vi "AssertEqual_Tests.vi"(11 "error in":errorcluster) -> (15 "error out":errorcluster)   [LabVIEW 2016, in "DronaTest.lvlib"]
uses:
  DronaTest.lvlib
  APIs/Assert/AssertControlValue/Equal.vi
  <vilib>/addons/_JKI Toolkits/Caraya/classes/Assert/Assert Equal Value_Variant.vi
  <vilib>/addons/_JKI Toolkits/Caraya/classes/Assert/Assert Error.vi
  <vilib>/addons/_JKI Toolkits/Caraya/classes/Test/Test.lvclass
  Drona.lvlib
  <vilib>/addons/_JKI Toolkits/Caraya/classes/Assert/Assert.lvclass
  APIs/Assert/AssertControlValue/AssertControlValue.lvlib
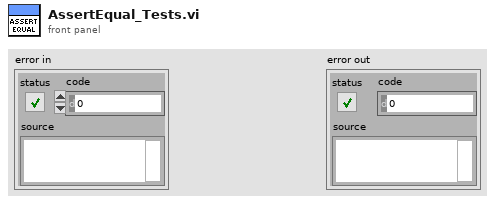
[diagram p1: front panel]
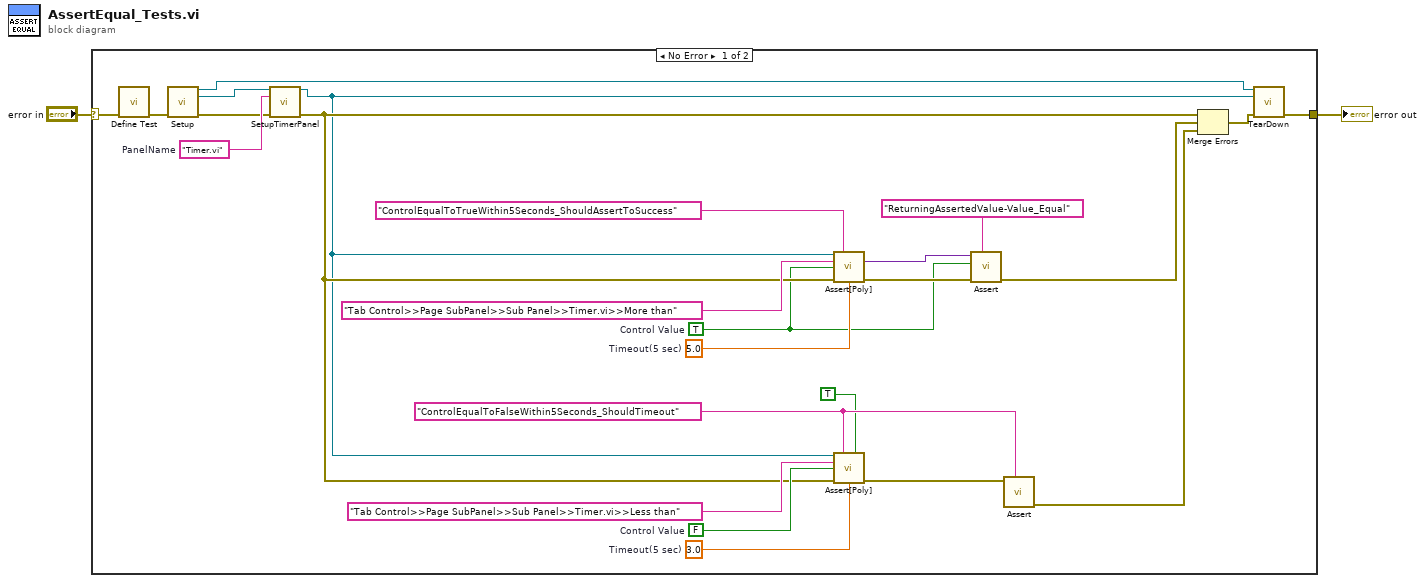
[diagram p0: block diagram]
diagram:
  n1 = case shown="No Error" "error in" {
    selector: "error in" -> [w27 w28]
    tunnel: [w12 w28] -> w1
    frame No Error {
      w17 = "Timer.vi"  # PanelName
      w26 = FALSE  # Control Value
      w23 = 3.0  # Timeout(5 sec)
      w22 = "ControlEqualToFalseWithin5Seconds_ShouldTimeout" ("string")
      w24 = 5.0  # Timeout(5 sec)
      w4 = TRUE  # Control Value
      n2 = call <vilib>:"Define Test.vi"("error in (no error)"=w27) -> ("error out"=w14:errorcluster)  [unwired: 9 in, 1 out]
      n3 = call "Setup.vi"("error in (no error)"=w14) -> ("Application Ref"=w11:refnum<vi>, "VI out"=w15:refnum<vi>, "error out"=w16:errorcluster)  [unwired: 12 in]
      n4 = call "SetupTimerPanel.vi"("VI in"=w15, "Item Name"=w17, "error in (no error)"=w16) -> ("VI out"=w9:refnum<vi>, "error out"=w10:errorcluster)  [unwired: 11 in]
      n5 = call-poly "Assert[Poly].vi"("VI Reference In"=w9, "Test Label"="ControlEqualToTrueWithin5Seconds_ShouldAssertToSuccess" ("string"), "Control Path"="Tab Control>>Page SubPanel>>Sub Panel>>Timer.vi>>More than", "Control Value"=w4, "Error In"=w10, "Timeout(5 sec)"=w24) -> ("Asserted Value"=w5:variant, "Error Out"=w7:errorcluster)  [unwired: 7 in, 1 out]
      n6 = call-poly "Assert[Poly].vi"("VI Reference In"=w9, "Test Label"=w22, "Assert Only? (F)"=TRUE, "Control Path"="Tab Control>>Page SubPanel>>Sub Panel>>Timer.vi>>Less than", "Control Value"=w26, "Error In"=w10, "Timeout(5 sec)"=w23) -> ("Error Out"=w21:errorcluster)  [unwired: 6 in, 2 out]
      n7 = call-poly <vilib>:"Assert.vi"("Label"="ReturningAssertedValue-Value_Equal", "error in (no error)"=w7, "Y"=w4, "X"=w5) -> ("error out"=w6:errorcluster)  [unwired: 6 in, 1 out]
      n8 = call-poly <vilib>:"Assert.vi"("Label"=w22, "Error?"=w21) -> ("error out"=w18:errorcluster)  [unwired: 8 in, 1 out]
      n9 = Merge Errors(w10, w6, w18) -> (w13:errorcluster)
      n10 = call "TearDown.vi"("Application Ref"=w11, "VI in"=w9, "error in (no error)"=w13) -> ("error out"=w12:errorcluster)  [unwired: 12 in]
    }
    frame Error {
    }
  }
  "error out" <- w1
